vi "Write file.vi"(8 "error in (no error)":errorcluster, 11 "Graph data":T1) -> (0 "error out":errorcluster)   [LabVIEW 2020]
uses:
  <vilib>/Utility/file.llb/Write Delimited Spreadsheet (string).vi
  <vilib>/Utility/sysdir.llb/System Directory Type.ctl
  controls/Graph data --typedef.ctl
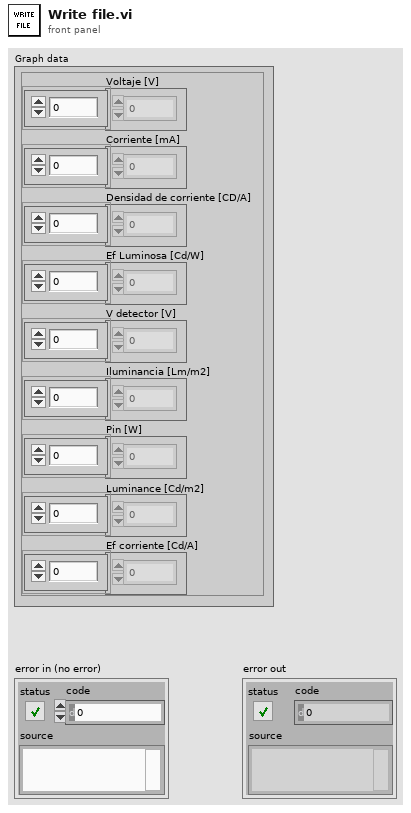
[diagram p1: front panel]
types:
  T1 = typedef "Graph data --typedef.ctl" = cluster{"Voltaje [V]":dbl[], "Corriente [mA]":dbl[], "Densidad de corriente [CD/A]":dbl[], "Ef Luminosa [Cd/W]":dbl[], "V detector [V]":dbl[], "Iluminancia [Lm/m2]":dbl[], "Pin [W]":dbl[], "Luminance [Cd/m2]":dbl[], "Ef corriente [Cd/A]":dbl[]}
  T2 = typedef "System Directory Type.ctl" = i32
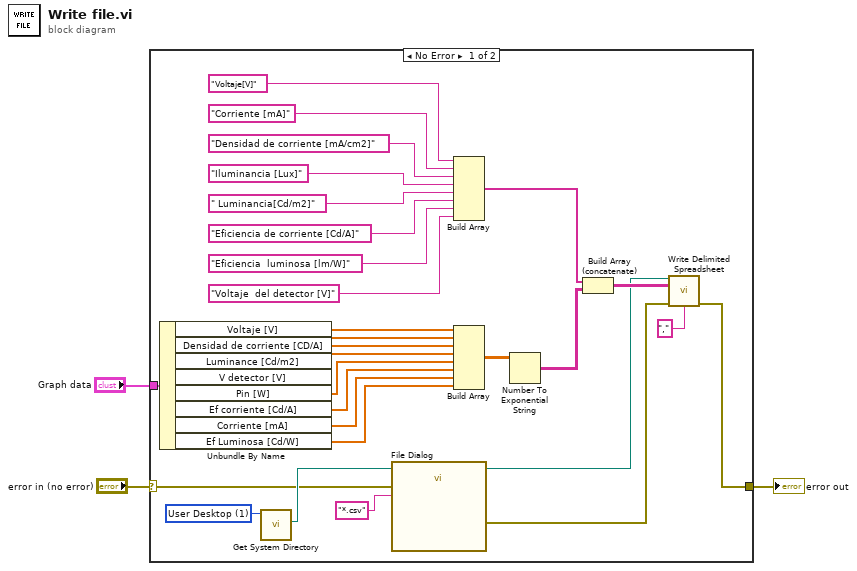
[diagram p0: block diagram]
diagram:
  n1 = case shown="No Error" "error in (no error)" {
    selector: "error in (no error)" -> [w7 w33]
    tunnel: "Graph data" -> [w28 _]
    tunnel: [w11 w33] -> w2
    frame No Error {
      w10 = T2 1 items=["User Home"=0, "User Desktop"=1, "User Documents"=2, "User Application Data"=3, "User Preferences"=4, "User Temporary"=5, "Public Documents"=6, "Public Application Data"=7, "Public Preferences"=8, "Public Cache"=13, "System Core Libraries"=9, "System Installed Libraries"=10, "Application Files"=11, "Boot Volume Root"=12] ("system directory type")
      n2 = Unbundle By Name(w28) -> ("Voltaje [V]"=w29:dbl[], "Densidad de corriente [CD/A]"=w30:dbl[], "Luminance [Cd/m2]"=w31:dbl[], "V detector [V]"=w32:dbl[], "Pin [W]"=w19:dbl[], "Ef corriente [Cd/A]"=w18:dbl[], "Corriente [mA]"=w17:dbl[], "Ef Luminosa [Cd/W]"=w16:dbl[])
      n3 = call <vilib>:"Get System Directory.vi"("system directory type"=w10) -> ("system directory"=w9:path)  [unwired: 10 in]
      n4 = call "File Dialog"("start path"=w9, "error in"=w7, "pattern (all files)"="*.csv") -> ("selected path"=w8:path, "error out"=w5:errorcluster)  [unwired: 9 in, 2 out]
      n5 = Build Array("Voltaje[V]", "Corriente [mA]", "Densidad de corriente [mA/cm2]", "Iluminancia [Lux]", " Luminancia[Cd/m2]", "Eficiencia de corriente [Cd/A]", "Eficiencia  luminosa [lm/W]", "Voltaje  del detector [V]") -> (w14:string[])
      n6 = Build Array(w29, w30, w31, w32, w19, w18, w17, w16) -> (w15:dbl[][])
      n7 = Number To Exponential String(number=w15) -> (E-format string=w13:string[][])  [unwired: 1 in, 2 out]
      n8 = Build Array (concatenate)(w14, w13) -> (w12:string[][])
      n9 = call-poly <vilib>:"Write Delimited Spreadsheet.vi"("file path (dialog if empty)"=w8, "2D data"=w12, "error in (no error)"=w5, "delimiter (\\t)"="," ("delimiter (\\t)")) -> ("error out"=w11:errorcluster)  [unwired: 10 in, 1 out]
    }
    frame Error {
    }
  }
  "error out" <- w2
